vi "Items_Collect.vi"(0 "State":T1={"Tick"=0, "Phase"=0, "PhaseTicks"=0, "Level"=1, "Room"=0, "X10"=0, "Y10"=0, "VY10"=0, "Mode"=0, "Facing"=0, "Run"=0, "Vert"=0, "StandY"=0, "EntryX10"=0, "EntryY10"=0, "EntryMode"=0, "Lives"=4, "Score"=0, "NextLife"=10000, "KeyR"=0, "KeyB"=0, "KeyY"=0, "Torch"=FALSE, "FloorPhase"=0, "Dead"=FALSE, "LevelStart"=FALSE, "Quit"=FALSE, "Sound"=0, "Seed"=12345, "DemoStep"=0, "Tiles"=[], "World"=[], "Enemies"=[], "Highscores"=[], "Name"=[0, 0, 0], "Cursor"=0}, 11 "error in":errorcluster) -> (4 "State out":T1={"Tick"=0, "Phase"=0, "PhaseTicks"=0, "Level"=1, "Room"=0, "X10"=0, "Y10"=0, "VY10"=0, "Mode"=0, "Facing"=0, "Run"=0, "Vert"=0, "StandY"=0, "EntryX10"=0, "EntryY10"=0, "EntryMode"=0, "Lives"=4, "Score"=0, "NextLife"=10000, "KeyR"=0, "KeyB"=0, "KeyY"=0, "Torch"=FALSE, "FloorPhase"=0, "Dead"=FALSE, "LevelStart"=FALSE, "Quit"=FALSE, "Sound"=0, "Seed"=12345, "DemoStep"=0, "Tiles"=[], "World"=[], "Enemies"=[], "Highscores"=[], "Name"=[0, 0, 0], "Cursor"=0}, 15 "error out":errorcluster)   [LabVIEW 2020, in "GH_Engine.lvlib"]
doc: "Collects the objects Claude touches (four points of his body): coin +100, gold hoard +500, key +200 and one key of its colour, torch +500 and light in all rooms. The tile becomes empty, the matching sound bit is set."
uses:
  GH_Engine.lvlib
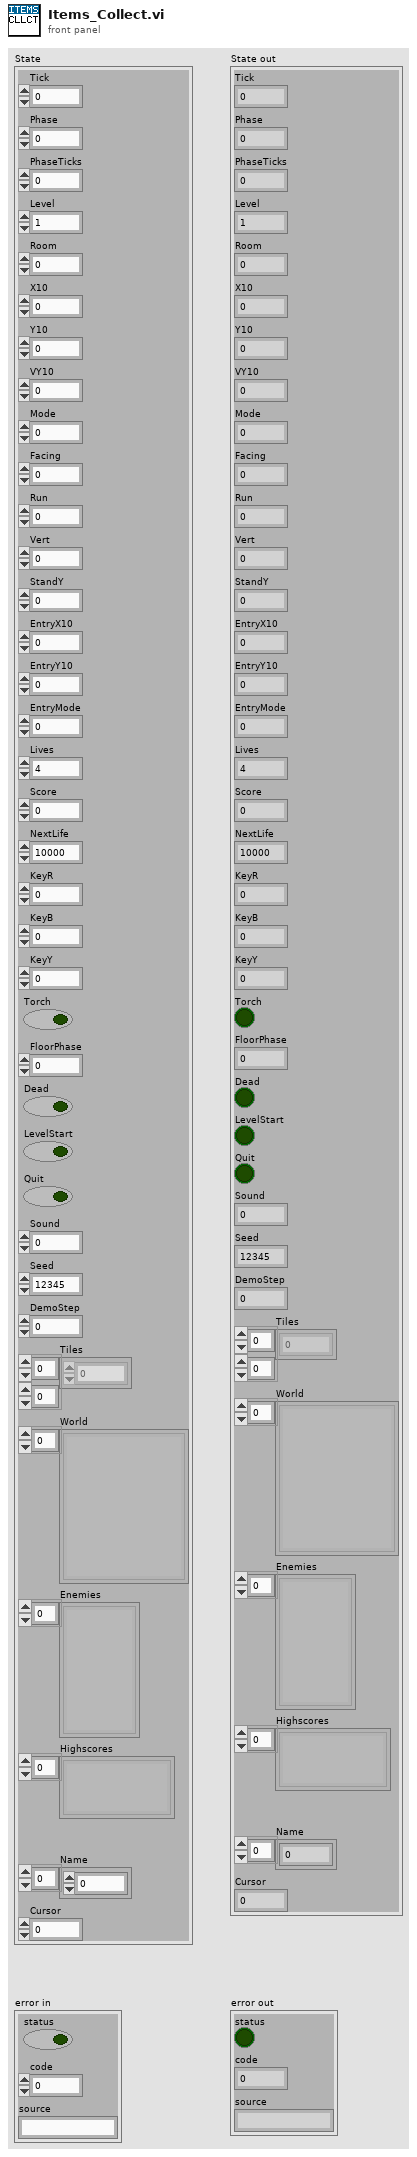
[diagram p1: front panel]
types:
  T1 = cluster{"Tick":u32, "Phase":i32, "PhaseTicks":i32, "Level":i32, "Room":i32, "X10":i32, "Y10":i32, "VY10":i32, "Mode":i32, "Facing":i32, "Run":i32, "Vert":i32, "StandY":i32, "EntryX10":i32, "EntryY10":i32, "EntryMode":i32, "Lives":i32, "Score":i32, "NextLife":i32, "KeyR":i32, "KeyB":i32, "KeyY":i32, "Torch":bool, "FloorPhase":i32, "Dead":bool, "LevelStart":bool, "Quit":bool, "Sound":i32, "Seed":u32, "DemoStep":i32, "Tiles":u8[][], "World":cluster{"ID":string, "Depth":i32, "Column":i32, "Tiles":u8[][]}[], "Enemies":cluster{"Kind":i32, "X10":i32, "Y10":i32, "Dir":i32, "Mode":i32}[], "Highscores":cluster{"Score":i32, "Name":string}[], "Name":i32[], "Cursor":i32}
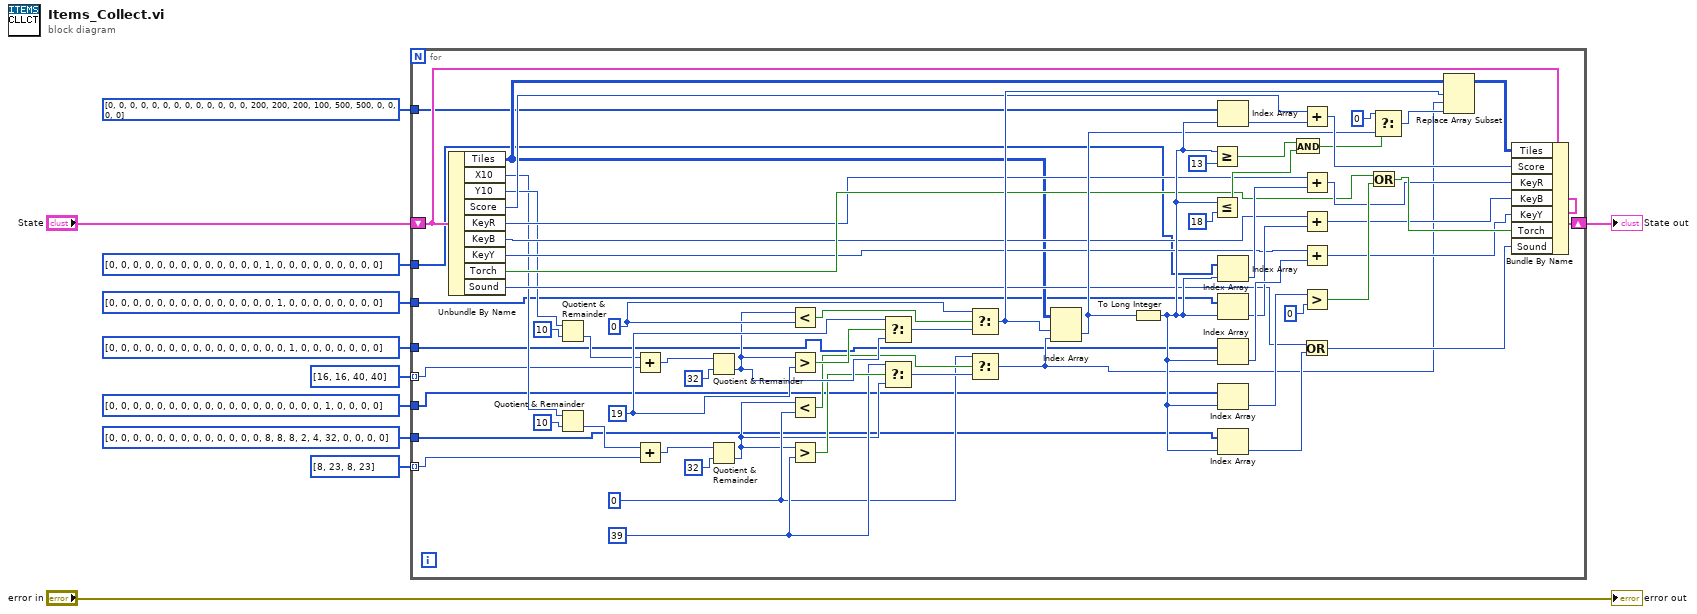
[diagram p0: block diagram]
diagram:
  n1 = for {
    tunnel: i32[] [8, 23, 8, 23] ("Probe X") -> [w12] mode=indexing
    tunnel: i32[] [16, 16, 40, 40] ("Probe Y") -> [w13] mode=indexing
    tunnel: i32[] [0, 0, 0, 0, 0, 0, 0, 0, 0, 0, 0, 0, 0, 200, 200, 200, 100, 500, 500, 0, 0, 0, 0] ("Points") -> [w14]
    tunnel: i32[] [0, 0, 0, 0, 0, 0, 0, 0, 0, 0, 0, 0, 0, 1, 0, 0, 0, 0, 0, 0, 0, 0, 0] ("Red key") -> [w15]
    tunnel: i32[] [0, 0, 0, 0, 0, 0, 0, 0, 0, 0, 0, 0, 0, 0, 1, 0, 0, 0, 0, 0, 0, 0, 0] ("Blue key") -> [w16]
    tunnel: i32[] [0, 0, 0, 0, 0, 0, 0, 0, 0, 0, 0, 0, 0, 0, 0, 1, 0, 0, 0, 0, 0, 0, 0] ("Yellow key") -> [w17]
    tunnel: i32[] [0, 0, 0, 0, 0, 0, 0, 0, 0, 0, 0, 0, 0, 0, 0, 0, 0, 0, 1, 0, 0, 0, 0] ("Torch") -> [w18]
    tunnel: i32[] [0, 0, 0, 0, 0, 0, 0, 0, 0, 0, 0, 0, 0, 8, 8, 8, 2, 4, 32, 0, 0, 0, 0] ("Sound") -> [w19]
    shift-right: [w21] -> w11
    shift-left: "State" -> [w20]
    w48 = 19
    w47 = 0
    w37 = 39
    w36 = 0
    n2 = Unbundle By Name(w20) -> ("Tiles"=w22:u8[][], "X10"=w23:i32, "Y10"=w24:i32, "Score"=w25:i32, "KeyR"=w26:i32, "KeyB"=w27:i32, "KeyY"=w28:i32, "Torch"=w29:bool, "Sound"=w30:i32)
    n3 = Quotient & Remainder(x=w24, y=10) -> (floor(x/y)=w43:i32)  [unwired: 1 out]
    n4 = Quotient & Remainder(x=w23, y=10) -> (floor(x/y)=w32:i32)  [unwired: 1 out]
    n5 = Add(x=w43, y=w13) -> (x+y=w44:i32)
    n6 = Add(x=w32, y=w12) -> (x+y=w33:i32)
    n7 = Quotient & Remainder(x=w44, y=32) -> (floor(x/y)=w46:i32)  [unwired: 1 out]
    n8 = Quotient & Remainder(x=w33, y=32) -> (floor(x/y)=w35:i32)  [unwired: 1 out]
    n9 = Less?(x=w46, y=w47) -> (x < y?=w49:bool)
    n10 = Greater?(x=w46, y=w48) -> (0:w50:bool)
    n11 = Less?(x=w35, y=w36) -> (x < y?=w38:bool)
    n12 = Greater?(x=w35, y=w37) -> (0:w39:bool)
    n13 = Select(t=w48, s=w50, f=w46) -> (s? t:f=w51:i32)
    n14 = Select(t=w37, s=w39, f=w35) -> (s? t:f=w40:i32)
    n15 = Select(t=w47, s=w49, f=w51) -> (s? t:f=w52:i32)
    n16 = Select(t=w36, s=w38, f=w40) -> (s? t:f=w41:i32)
    n17 = Index Array(array=w22, index (row)=w52, index (col)=w41) -> (element=w53:u8)
    n18 = To Long Integer(number=w53) -> (32bit integer=w54:i32)
    n19 = Greater Or Equal?(x=w54, y=13) -> (x >= y?=w56:bool)
    n20 = Less Or Equal?(x=w54, y=18) -> (x <= y?=w58:bool)
    n21 = Index Array(array=w14, index=w54) -> (element=w63:i32)
    n22 = Index Array(array=w15, index=w54) -> (element=w65:i32)
    n23 = Index Array(array=w16, index=w54) -> (element=w67:i32)
    n24 = Index Array(array=w17, index=w54) -> (element=w69:i32)
    n25 = Index Array(array=w18, index=w54) -> (element=w71:i32)
    n26 = Index Array(array=w19, index=w54) -> (element=w75:i32)
    n27 = And(x=w56, y=w58) -> (x .and. y?=w59:bool)
    n28 = Add(x=w25, y=w63) -> (x+y=w64:i32)
    n29 = Add(x=w26, y=w65) -> (x+y=w66:i32)
    n30 = Add(x=w27, y=w67) -> (x+y=w68:i32)
    n31 = Add(x=w28, y=w69) -> (x+y=w70:i32)
    n32 = Greater?(x=w71, y=0) -> (0:w73:bool)
    n33 = Or(x=w30, y=w75) -> (x .or. y?=w76:i32)
    n34 = Or(x=w29, y=w73) -> (x .or. y?=w74:bool)
    n35 = Select(t=u8 0, s=w59, f=w53) -> (s? t:f=w61:u8)
    n36 = Replace Array Subset(array=w22, new element=w61, index (row)=w52, index (col)=w41) -> (w62:u8[][])
    n37 = Bundle By Name(cluster=w20, "Tiles"=w62, "Score"=w64, "KeyR"=w66, "KeyB"=w68, "KeyY"=w70, "Torch"=w74, "Sound"=w76) -> (w21:T1)
  }
  "State out" <- w11
  "error out" <- "error in"
